vi "Mark Precision.vi"(8 "error in (no error)":errorcluster caption="에러 입력(에러 없음)", 11 "Instrument Manager 입력":refnum<class "Instrument Manager.lvclass">) -> (0 "error out":errorcluster caption="에러 출력", 2 "Marker Value":T1 {"X-axis" format="%#_6p"}, 3 "Instrument Manager 출력":refnum<class "Instrument Manager.lvclass">)   [LabVIEW 2023, in "Instrument Manager.lvclass"]
uses:
  Instrument Manager.lvclass
  Module/Spectrum Analyzer/TYPE DEFINITION/TYPE Marker Value.ctl
  Instrument Manager.lvclass/Instrument Manager.ctl
  Module/Spectrum Analyzer/Spectrum Analyzer.lvlib
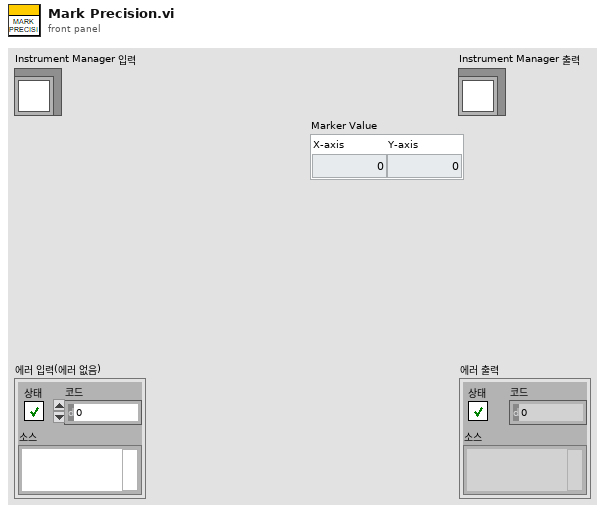
[diagram p1: front panel]
types:
  T1 = typedef "Spectrum Analyzer.lvlib/TYPE Marker Value.ctl" = cluster{"X-axis":dbl, "Y-axis":dbl}
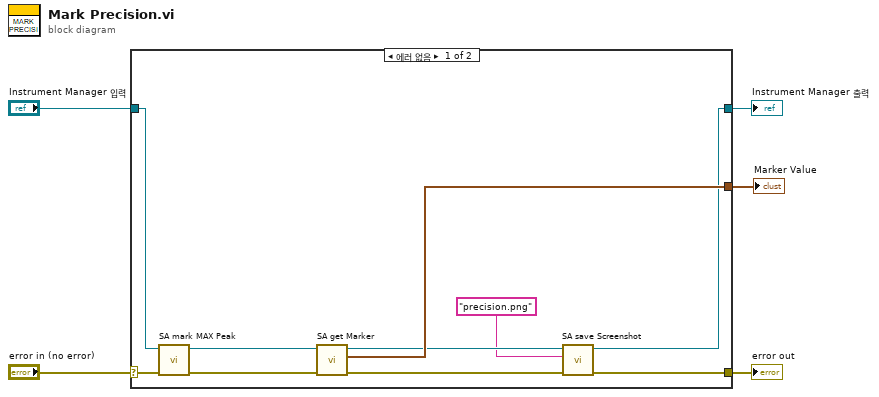
[diagram p0: block diagram]
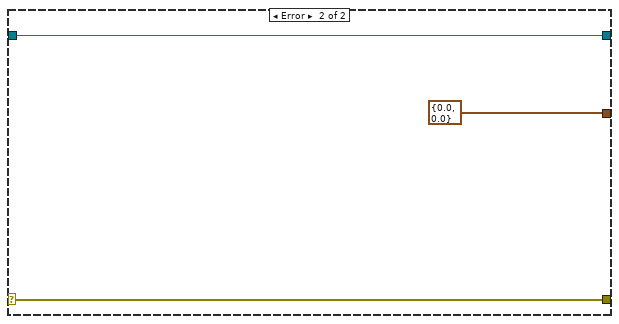
[diagram p2: hidden frame]
diagram:
  n1 = case shown="에러 없음" "error in (no error)" {
    selector: "error in (no error)" -> [w15 w18]
    tunnel: [w9 w18] -> w4
    tunnel: [w7 w17] -> w2
    tunnel: "Instrument Manager 입력" -> [w13 w17]
    tunnel: [w11 T1 {"X-axis"=0.0, "Y-axis"=0.0} ("Marker Value")] -> w1
    frame No Error {
      n2 = call "SA mark MAX Peak.vi"("error in (no error)"=w15, "Instrument Manager 입력"=w13) -> ("error out"=w14:errorcluster, "Instrument Manager 출력"=w12:refnum<class "Instrument Manager.lvclass">)  [unwired: 8 in]
      n3 = call "SA get Marker.vi"("error in (no error)"=w14, "Instrument Manager 입력"=w12) -> ("error out"=w10:errorcluster, "Marker Value"=w11:T1, "Instrument Manager 출력"=w8:refnum<class "Instrument Manager.lvclass">)  [unwired: 7 in]
      n4 = call "SA save Screenshot.vi"("error in (no error)"=w10, "File Name"="precision.png", "Instrument Manager 입력"=w8) -> ("error out"=w9:errorcluster, "Instrument Manager 출력"=w7:refnum<class "Instrument Manager.lvclass">)  [unwired: 7 in]
    }
    frame Error {
    }
  }
  "error out" <- w4
  "Instrument Manager 출력" <- w2
  "Marker Value" <- w1
